vi "RemoteVI Call Hooks.vi"(0 "hooks":refnum<vi>, 1 "panel?":bool, 2 "mods":u8, 3 "VI name":string, 5 "origin":cluster{"x":i32, "y":i32}, 6 "tips in":string="tips []", 7 "splitters in":string="splitters []", 8 "bars in":T1(array[cluster]), 11 "error in":errorcluster) -> (4 "tips out":string, 9 "splitters out":string, 10 "bars out":T1(array[cluster]), 15 "error out":errorcluster)   [LabVIEW 2020, in "RemoteVI.lvlib"]
doc: "Runs RemoteVI Remote Hooks.vi in the other LabVIEW (hooks, opened there by RemoteVI Connect VI Server.vi) over VI Server: sets its controls (Set Control Value), runs it and waits (Run VI), and reads tips out, splitters out and bars out back (Get Control Value) when panel? is TRUE. One VI Server round trip per control, about a millisecond each on this computer. On an error the inputs pass through."
uses:
  RemoteVI.lvlib
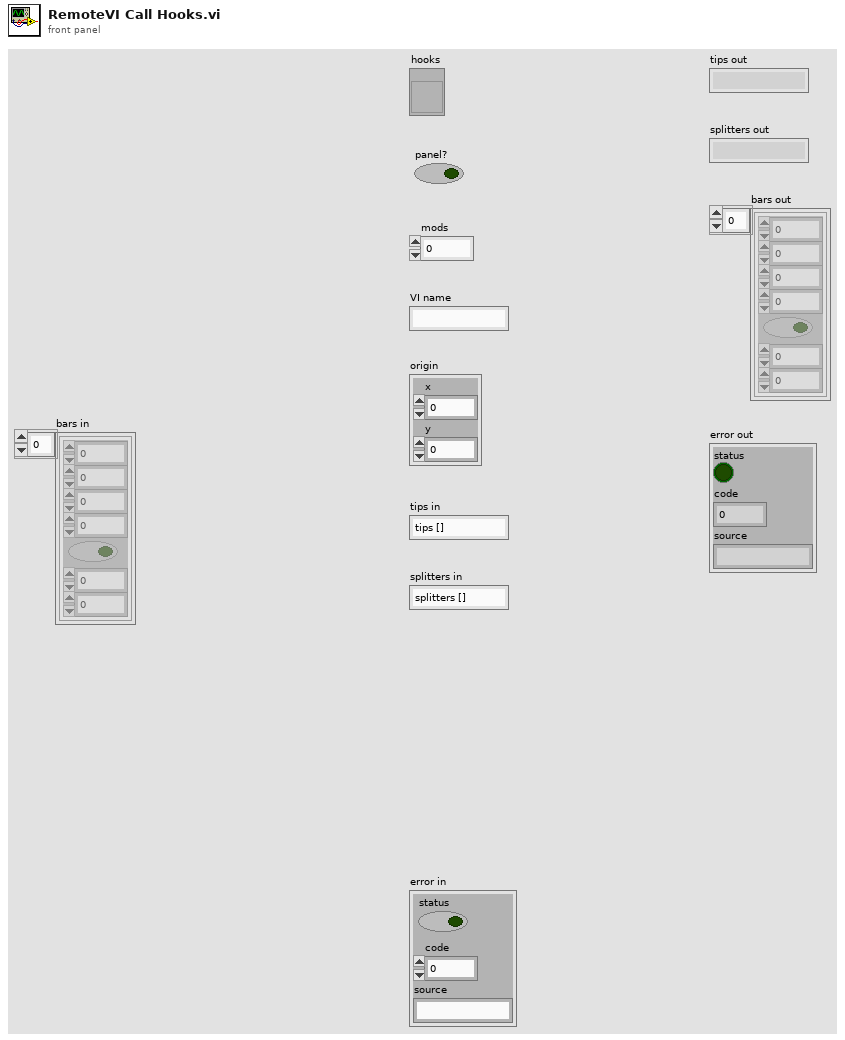
[diagram p1: front panel]
types:
  T1 = cluster{"x":i32, "y":i32, "w":i32, "h":i32, "vertical":bool, "min":i32, "max":i32}[]
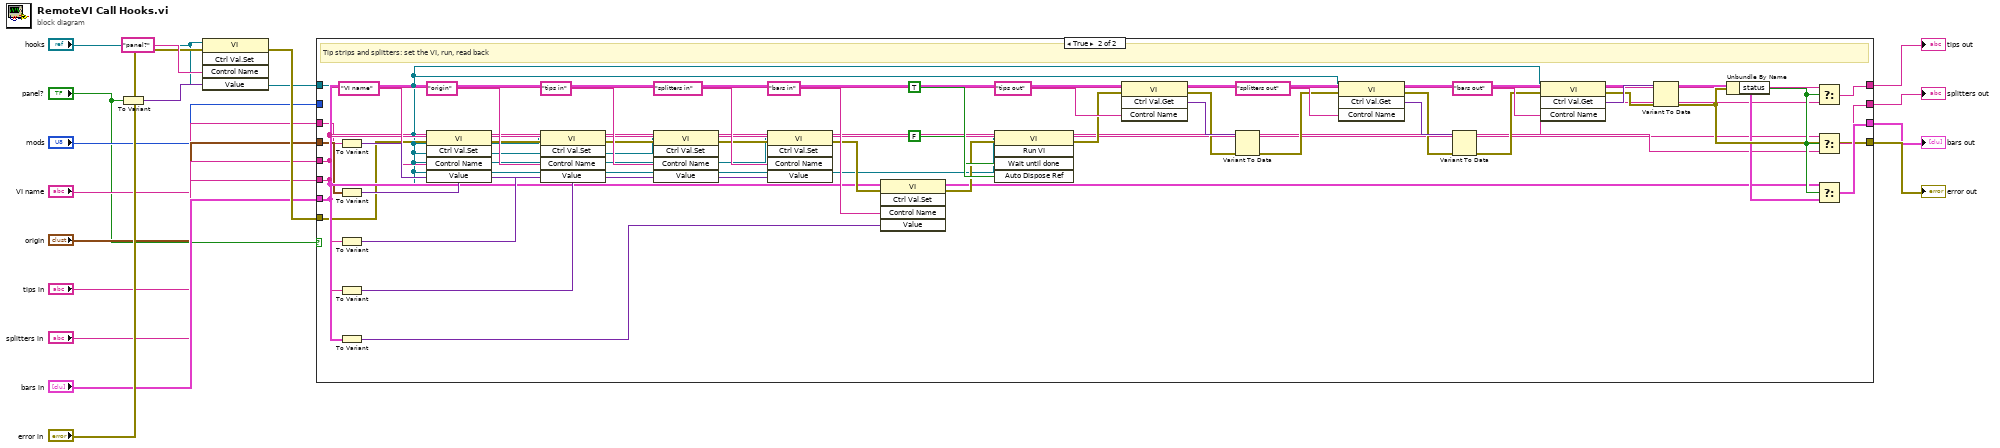
[diagram p0: block diagram]
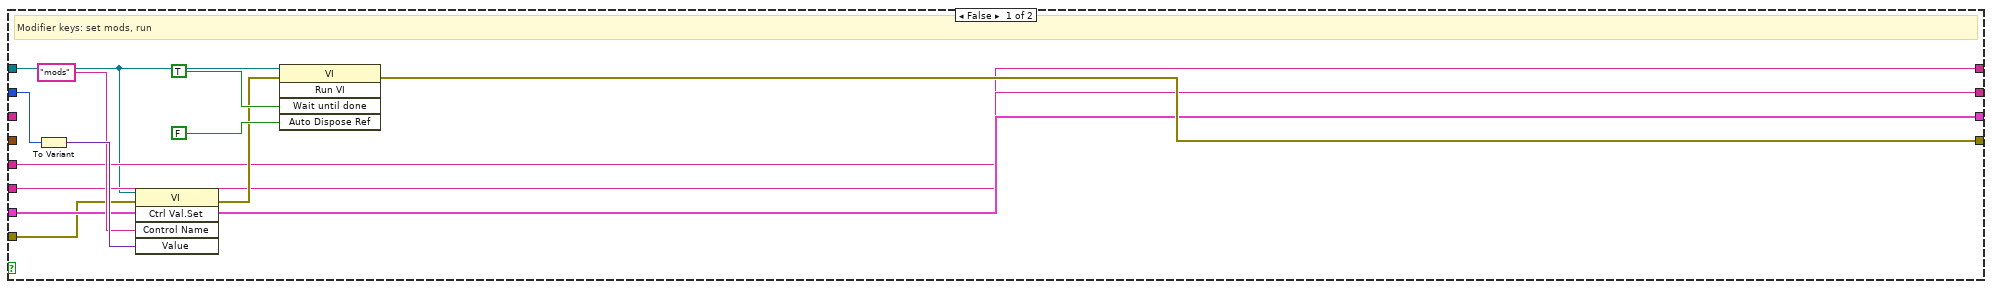
[diagram p2: hidden frame]
diagram:
  n1 = To Variant(anything="panel?") -> (Variant=w11:variant)
  n2 = invoke class="VI" method="Ctrl Val.Set"(reference="hooks", error in="error in", "Control Name"="panel?", "Value"=w11) -> (error out=w12:errorcluster)  [unwired: 1 in, 4 out]
  n3 = case shown="True" "panel?" {
    tunnel: "hooks" -> [w17 w29]
    tunnel: "mods" -> [w19 _]
    tunnel: "VI name" -> [_ w31]
    tunnel: "origin" -> [_ w32]
    tunnel: "tips in" -> [w20 w33]
    tunnel: "splitters in" -> [w21 w34]
    tunnel: "bars in" -> [w22 w35]
    tunnel: [w20 w70] -> w13
    tunnel: [w21 w71] -> w14
    tunnel: [w22 w72] -> w15
    tunnel: w12 -> [w18 w30]
    tunnel: [w28 w68] -> w16
    frame False {
      # "Modifier keys: set mods, run"
      n4 = To Variant(anything=w19) -> (Variant=w24:variant)
      n5 = invoke class="VI" method="Ctrl Val.Set"(reference=w17, error in=w18, "Control Name"="mods", "Value"=w24) -> (error out=w25:errorcluster)  [unwired: 1 in, 4 out]
      n6 = invoke class="VI" method="Run VI"(reference=w17, error in=w25, "Wait until done"=TRUE, "Auto Dispose Ref"=FALSE) -> (error out=w28:errorcluster)  [unwired: 1 in, 4 out]
    }
    frame True {
      # "Tip strips and splitters: set the VI, run, read back"
      n7 = To Variant(anything=w31) -> (Variant=w37:variant)
      n8 = To Variant(anything=w32) -> (Variant=w40:variant)
      n9 = To Variant(anything=w33) -> (Variant=w43:variant)
      n10 = To Variant(anything=w34) -> (Variant=w46:variant)
      n11 = To Variant(anything=w35) -> (Variant=w49:variant)
      n12 = invoke class="VI" method="Ctrl Val.Set"(reference=w29, error in=w30, "Control Name"="VI name", "Value"=w37) -> (error out=w38:errorcluster)  [unwired: 1 in, 4 out]
      n13 = invoke class="VI" method="Ctrl Val.Set"(reference=w29, error in=w38, "Control Name"="origin", "Value"=w40) -> (error out=w41:errorcluster)  [unwired: 1 in, 4 out]
      n14 = invoke class="VI" method="Ctrl Val.Set"(reference=w29, error in=w41, "Control Name"="tips in", "Value"=w43) -> (error out=w44:errorcluster)  [unwired: 1 in, 4 out]
      n15 = invoke class="VI" method="Ctrl Val.Set"(reference=w29, error in=w44, "Control Name"="splitters in", "Value"=w46) -> (error out=w47:errorcluster)  [unwired: 1 in, 4 out]
      n16 = invoke class="VI" method="Ctrl Val.Set"(reference=w29, error in=w47, "Control Name"="bars in", "Value"=w49) -> (error out=w50:errorcluster)  [unwired: 1 in, 4 out]
      n17 = invoke class="VI" method="Run VI"(reference=w29, error in=w50, "Wait until done"=TRUE, "Auto Dispose Ref"=FALSE) -> (error out=w53:errorcluster)  [unwired: 1 in, 4 out]
      n18 = invoke class="VI" method="Ctrl Val.Get"(reference=w29, error in=w53, "Control Name"="tips out") -> (error out=w55:errorcluster, "Get Control Value Variant"=w56:variant)  [unwired: 1 in, 2 out]
      n19 = Variant To Data(error in=w55, type=w33, Variant=w56) -> (data=w57:string, error out=w58:errorcluster)
      n20 = invoke class="VI" method="Ctrl Val.Get"(reference=w29, error in=w58, "Control Name"="splitters out") -> (error out=w60:errorcluster, "Get Control Value Variant"=w61:variant)  [unwired: 1 in, 2 out]
      n21 = Variant To Data(error in=w60, type=w34, Variant=w61) -> (data=w62:string, error out=w63:errorcluster)
      n22 = invoke class="VI" method="Ctrl Val.Get"(reference=w29, error in=w63, "Control Name"="bars out") -> (error out=w65:errorcluster, "Get Control Value Variant"=w66:variant)  [unwired: 1 in, 2 out]
      n23 = Variant To Data(error in=w65, type=w35, Variant=w66) -> (data=w67:T1, error out=w68:errorcluster)
      n24 = Unbundle By Name(w68) -> ("status"=w69:bool)
      n25 = Select(t=w33, s=w69, f=w57) -> (s? t:f=w70:string)
      n26 = Select(t=w34, s=w69, f=w62) -> (s? t:f=w71:string)
      n27 = Select(t=w35, s=w69, f=w67) -> (s? t:f=w72:T1)
    }
  }
  "tips out" <- w13
  "splitters out" <- w14
  "bars out" <- w15
  "error out" <- w16
